vi "Add Server Library to Project.vi"(8 "error in (no error)":errorcluster, 10 "Project Settings":T1) -> (0 "error out":errorcluster)   [LabVIEW 2019, in "gRPC Template Creation Utility.lvlib"]
uses:
  gRPC Template Creation Utility.lvlib
  TypeDefs/Project Settings.ctl
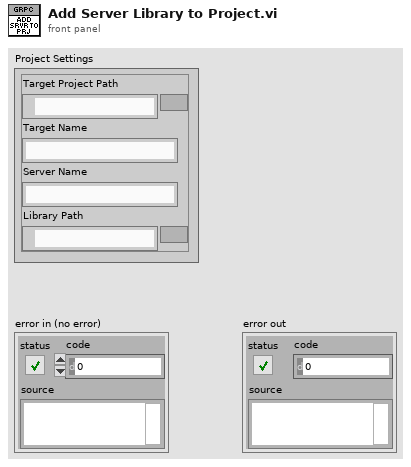
[diagram p1: front panel]
types:
  T1 = typedef "gRPC Template Creation Utility.lvlib/Project Settings.ctl" = cluster{"Target Project Path":path, "Target Name":string, "Server Name":string, "Library Path":path}
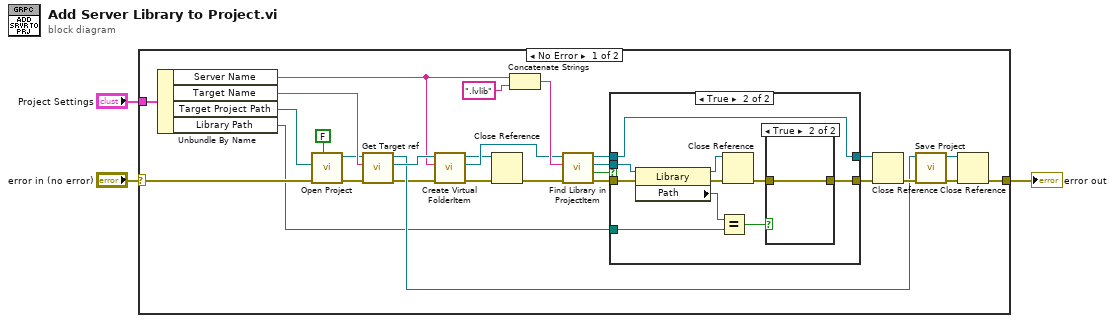
[diagram p0: block diagram]
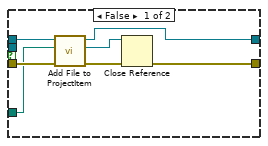
[diagram p2: hidden frame]
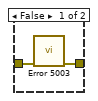
[diagram p3: hidden frame]
diagram:
  n1 = case shown="No Error" "error in (no error)" {
    selector: "error in (no error)" -> [w9 w52]
    tunnel: [w16 w52] -> w3
    tunnel: "Project Settings" -> [w11 _]
    frame No Error {
      n2 = Unbundle By Name(w11) -> ("Server Name"=w10:string, "Target Name"=w6:string, "Target Project Path"=w7:path, "Library Path"=w8:path)
      n3 = call "Open Project.vi"("Open Project Window ?"=FALSE, "error in (no error)"=w9, "Project Path in"=w7) -> ("error out"=w13:errorcluster, "Project out"=w4:refnum<vi>)  [unwired: 7 in]
      n4 = call "Get Target ref.vi"("error in (no error)"=w13, "Target Name"=w6, "Project in"=w4) -> ("error out"=w12:errorcluster, "Target ref out"=w15:refnum<vi>, "Project out"=w14:refnum<vi>)  [unwired: 6 in]
      n5 = call "Create Virtual FolderItem.vi"("error in (no error)"=w12, "Folder Name"=w10, "ProjectItem in"=w15) -> ("error out"=w22:errorcluster, "FolderItem reference out"=w23:refnum<vi>, "ProjectItem out"=w5:refnum<vi>)  [unwired: 5 in, 1 out]
      n6 = Close Reference(reference=w5, error in (no error)=w22) -> (error out=w19:errorcluster)
      n7 = Concatenate Strings(w10, ".lvlib" ("string")) -> (w25:string)
      n8 = call "Find Library in ProjectItem.vi"("error in (no error)"=w19, "Library Name"=w25, "ProjectItem in"=w23) -> ("error out"=w27:errorcluster, "Found?"=w26:bool, "Library out"=w29:refnum<vi>, "ProjectItem out"=w28:refnum<vi>)  [unwired: 5 in]
      n9 = case shown="True" w26 {
        tunnel: [w34 w46] -> w30
        tunnel: w27 -> [w35 w45]
        tunnel: w28 -> [w36 w39]
        tunnel: w29 -> [_ w44]
        tunnel: [w33 w39] -> w31
        tunnel: w8 -> [w32 w41]
        frame False {
          n10 = call "Add File to ProjectItem.vi"("error in (no error)"=w35, "File Path"=w32, "ProjectItem in"=w36) -> ("error out"=w37:errorcluster, "Added File ref"=w38:refnum<vi>, "ProjectItem out"=w33:refnum<vi>)  [unwired: 6 in]
          n11 = Close Reference(reference=w38, error in (no error)=w37) -> (error out=w34:errorcluster)
        }
        frame True {
          n12 = property class="Library"(reference=w44, error in=w45) -> (reference out=w42:refnum<vi>, error out=w40:errorcluster, "Path"=w48:path)
          n13 = Equal?(x=w48, y=w41) -> (x = y?=w47:bool)
          n14 = Close Reference(reference=w42, error in (no error)=w40) -> (error out=w43:errorcluster)
          n15 = case shown="True" w47 {
            tunnel: w43 -> [w50 w51]
            tunnel: [w49 w51] -> w46
            frame False {
              n16 = call "Error 5003.vi"("error in (no error)"=w50) -> ("error out"=w49:errorcluster)  [unwired: 10 in]
            }
            frame True {
            }
          }
        }
      }
      n17 = Close Reference(reference=w31, error in (no error)=w30) -> (error out=w20:errorcluster)
      n18 = call "Save Project.vi"("error in (no error)"=w20, "Project in"=w14) -> ("error out"=w18:errorcluster, "Project out"=w17:refnum<vi>)  [unwired: 8 in]
      n19 = Close Reference(reference=w17, error in (no error)=w18) -> (error out=w16:errorcluster)
    }
    frame Error {
    }
  }
  "error out" <- w3
